vi "Init HTTP.vi"(8 "error in (no error)":errorcluster, 11 "Hardware Info Module in":refnum<class "Hardware Info Module.lvclass">) -> (0 "error out":errorcluster, 3 "Hardware Info Module out":refnum<class "Hardware Info Module.lvclass">)   [LabVIEW 2020, in "Volatus.lvlib" / "Hardware Info Module.lvclass"]
uses:
  Hardware Info Module.lvclass
  Hardware Info Module.lvclass/Hardware Info Module.ctl
  Module/Module.lvclass
  VolatusAPI/VolatusAPI.lvclass
  HardwareHTTPController/HardwareHTTPController.lvclass
  C:/dev/lv20CE/relink/lv-volatus/Volatus/Module/Module.lvclass
  C:/dev/lv20CE/relink/lv-volatus/Volatus/Hardware Info Module/Hardware Info Module.lvclass
  C:/dev/lv20CE/relink/lv-http-server/HTTP Server/Controller/Controller.lvclass
  C:/dev/lv20CE/relink/lv-http-server/HTTP Server/Handler/Handler.lvclass
  C:/dev/lv20CE/relink/lv-volatus/Volatus/HardwareHTTPController/HardwareHTTPController.lvclass
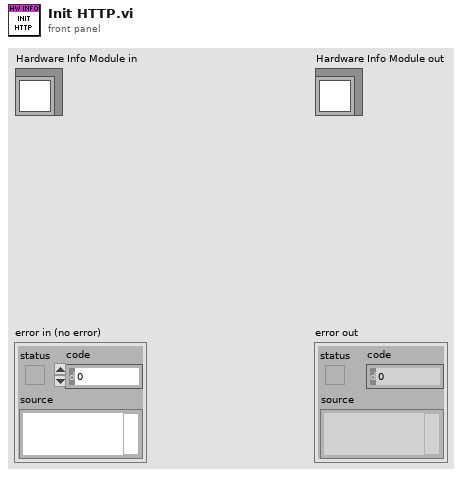
[diagram p1: front panel]
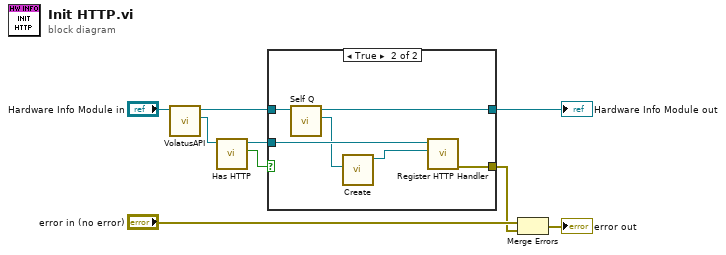
[diagram p0: block diagram]
diagram:
  n1 = call "VolatusAPI.vi"("Module in"="Hardware Info Module in") -> ("VolatusAPI"=w7:refnum<class "VolatusAPI.lvclass">, "Module out"=w5:refnum<class "Hardware Info Module.lvclass">)  [unwired: 9 in]
  n2 = call "Has HTTP.vi"("VolatusAPI in"=w7) -> ("Has HTTP"=w4:bool, "VolatusAPI out"=w3:refnum<class "VolatusAPI.lvclass">)  [unwired: 9 in]
  n3 = case shown="True" w4 {
    tunnel: [w10 w16] -> w8
    tunnel: w5 -> [w10 w15]
    tunnel: w3 -> [_ w14]
    tunnel: [_ w11] -> w1
    frame False {
    }
    frame True {
      n4 = call "Self Q.vi"("Module in"=w15) -> ("Self Q"=w13:refnum<class "MessageQ.lvclass">, "Module out"=w16:refnum<class "Hardware Info Module.lvclass">)  [unwired: 9 in]
      n5 = call "Create.vi"("MsgQ"=w13) -> ("HardwareHTTPController out"=w12:refnum<class "HardwareHTTPController.lvclass">)  [unwired: 9 in, 1 out]
      n6 = call "Register HTTP Handler.vi"("Handler"=w12, "VolatusAPI in"=w14) -> ("error out"=w11:errorcluster)  [unwired: 8 in, 1 out]
    }
  }
  "Hardware Info Module out" <- w8
  n7 = Merge Errors("error in (no error)", w1) -> (→"error out":errorcluster)
